vi "Violet--constant.vi"() -> (1 "Violet":u32(colorbox))   [LabVIEW 2018, in "Band Colors.lvlib"]
doc: "Provides the RGB color value for violet.\n\nThe VI converts the RGB components (148, 0, 211) into a LabVIEW color value and returns it through <b>Violet</b>."
uses:
  Band Colors.lvlib
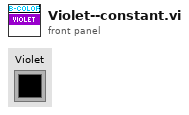
[diagram p1: front panel]
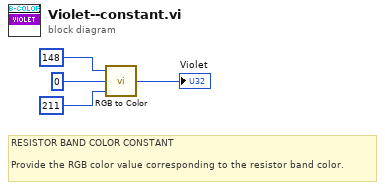
[diagram p0: block diagram]
diagram:
  # "RESISTOR BAND COLOR CONSTANT\n\nProvide the RGB color value corresponding to the resistor band color."
  n1 = call <vilib>:"RGB to Color.vi"("B"=u8 211, "G"=u8 0, "R"=u8 148) -> ("Color"=→"Violet":u32)
